vi "Test MQTT-2.2.2-2.vi"(8 "error in (no error)":errorcluster, 11 "Connection Config":refnum<class "Connection.lvclass">) -> (0 "error out":errorcluster, 3 "Connection Config dup":refnum<class "Connection.lvclass">)   [LabVIEW 2013]
uses:
  <vilib>/addons/_JKI Toolkits/Caraya/classes/Test/Test.lvclass
  <vilib>/LabVIEW Open Source Project/MQTT Control Packets/Control Packets/CONNECT/CONNECT.lvclass
  <vilib>/LabVIEW Open Source Project/MQTT Control Packets/Control Packets/ControlPacket/ControlPacket.lvclass
  <vilib>/addons/_JKI Toolkits/Caraya/classes/Assert/Assert.lvclass
  <vilib>/LabVIEW Open Source Project/Connection/Connection/Connection.lvclass
  <vilib>/LabVIEW Open Source Project/MQTT Connection/MQTT_Connection/Connection/Connection.lvclass
panel:
  out "connected":bool
  out "error out 2":errorcluster
  out "timed out":bool
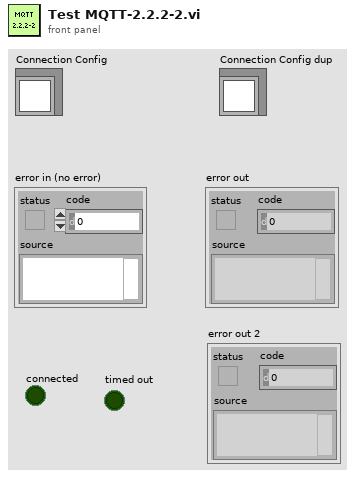
[diagram p1: front panel]
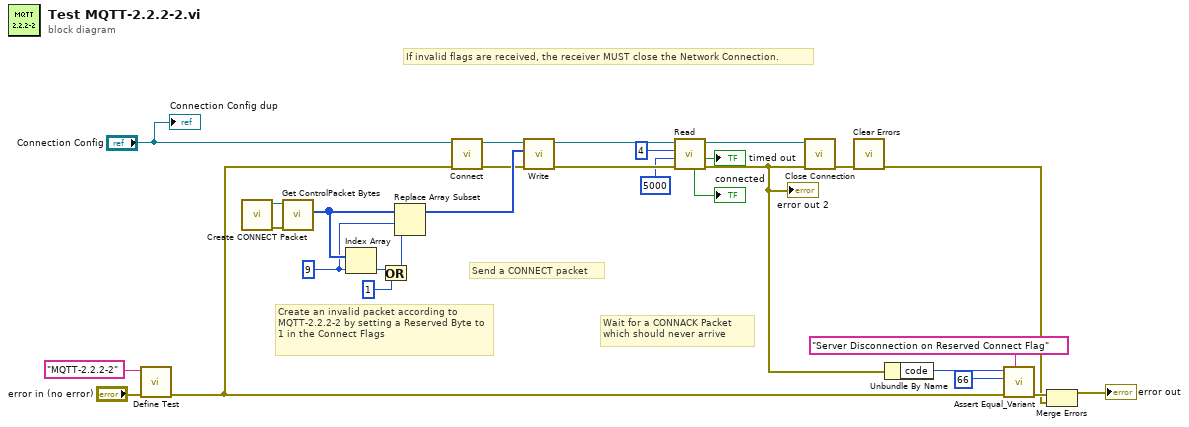
[diagram p0: block diagram]
diagram:
  w19 = 9 ("index")
  # "Wait for a CONNACK Packet\nwhich should never arrive"
  # "Create an invalid packet according to MQTT-2.2.2-2 by setting a Reserved Byte to 1 in the Connect Flags"
  # "Send a CONNECT packet"
  # "If invalid flags are received, the receiver MUST close the Network Connection."
  n1 = call <vilib>:"Define Test.vi"("error in (no error)"="error in (no error)", "Label (VI Title)"="MQTT-2.2.2-2") -> ("error out"=w3:errorcluster)  [unwired: 9 in]
  n2 = call <vilib>:"Create CONNECT Packet.vi"() -> ("error out"=w26:errorcluster, "CONNECT"=w27:refnum<class "CONNECT.lvclass">)  [unwired: 9 in, 1 out]
  n3 = call <vilib>:"Get ControlPacket Bytes.vi"("error in (no error)"=w26, "ControlPacket"=w27) -> ("Bytes Stream"=w21:u8[])  [unwired: 6 in, 3 out]
  n4 = Index Array(array=w21, index=w19) -> (element=w23:u8)
  n5 = Or(x=w23, y=u8 1) -> (x .or. y?=w18:u8)
  n6 = Replace Array Subset(array=w21, new element=w18, index=w19) -> (w20:u8[])
  n7 = call <vilib>:"Connect.vi"("error in (no error)"=w3, "Connection in"="Connection Config") -> ("error out"=w6:errorcluster, "Connection out"=w7:refnum<class "Connection.lvclass">)  [unwired: 8 in]
  n8 = call <vilib>:"Write.vi"("error in (no error)"=w6, "Bytes"=w20, "Connection in"=w7) -> ("error out"=w24:errorcluster, "Connection"=w25:refnum<class "Connection.lvclass">)  [unwired: 7 in]
  n9 = call <vilib>:"Read.vi"("error in (no error)"=w24, "timeout (2000 ms)"=5000 ("timeout ms (25000)"), "bytes to read (100)"=4 ("bytes to read"), "TCPConnection in"=w25) -> ("error out"=w9:errorcluster, "timed out"=→"timed out":bool, "TCPConnection out"=w17:refnum<class "Connection.lvclass">, "connected"=→"connected":bool)  [unwired: 3 in, 1 out]
  "error out 2" <- w9
  n10 = call <vilib>:"Close Connection.vi"("error in (no error)"=w9, "Connection in"=w17) -> ("error out"=w12:errorcluster)  [unwired: 8 in, 1 out]
  n11 = call <vilib>:"Clear Errors.vi"("error in (no error)"=w12) -> ("error out"=w2:errorcluster)  [unwired: 6 in]
  n12 = Unbundle By Name(w9) -> ("code"=w14:i32)
  n13 = call <vilib>:"Assert Equal_Variant.vi"("Label"="Server Disconnection on Reserved Connect Flag", "error in (no error)"=w3, "Y"=66 ("code"), "X"=w14) -> ("error out"=w16:errorcluster)  [unwired: 7 in]
  n14 = Merge Errors(w16, w2) -> (→"error out":errorcluster)
  "Connection Config dup" <- "Connection Config"
